vi "TestProcess.vi"(0 "VI Reference In":refnum<vi>, 5 "Wash Option":string, 7 "Car Position":u8=1, 9 "Elapsed Time":dbl=5.0, 11 "error in":errorcluster, 13 "Same Position?":bool) -> (4 "VI Reference Out":refnum<vi>, 15 "error out":errorcluster)   [LabVIEW 2016, in "CarWashTest.lvlib"]
doc: "Test Process function"
uses:
  CarWashTest.lvlib
  APIs/Assert/AssertControlValue/False.vi
  APIs/Assert/AssertControlValue/True.vi
  APIs/Stimulus/ControlValue/SetValueAuto.vi
  APIs/Assert/AssertControlValue/Equal.vi
  APIs/Assert/AssertControlValue/AlmostEqual.vi
  <vilib>/addons/_JKI Toolkits/Caraya/classes/Test/Test.lvclass
  Drona.lvlib
  APIs/Assert/AssertControlValue/AssertControlValue.lvlib
  APIs/Stimulus/ControlValue/ControlValue.lvlib
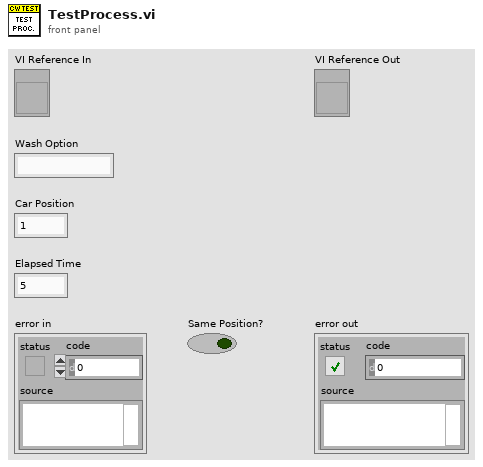
[diagram p1: front panel]
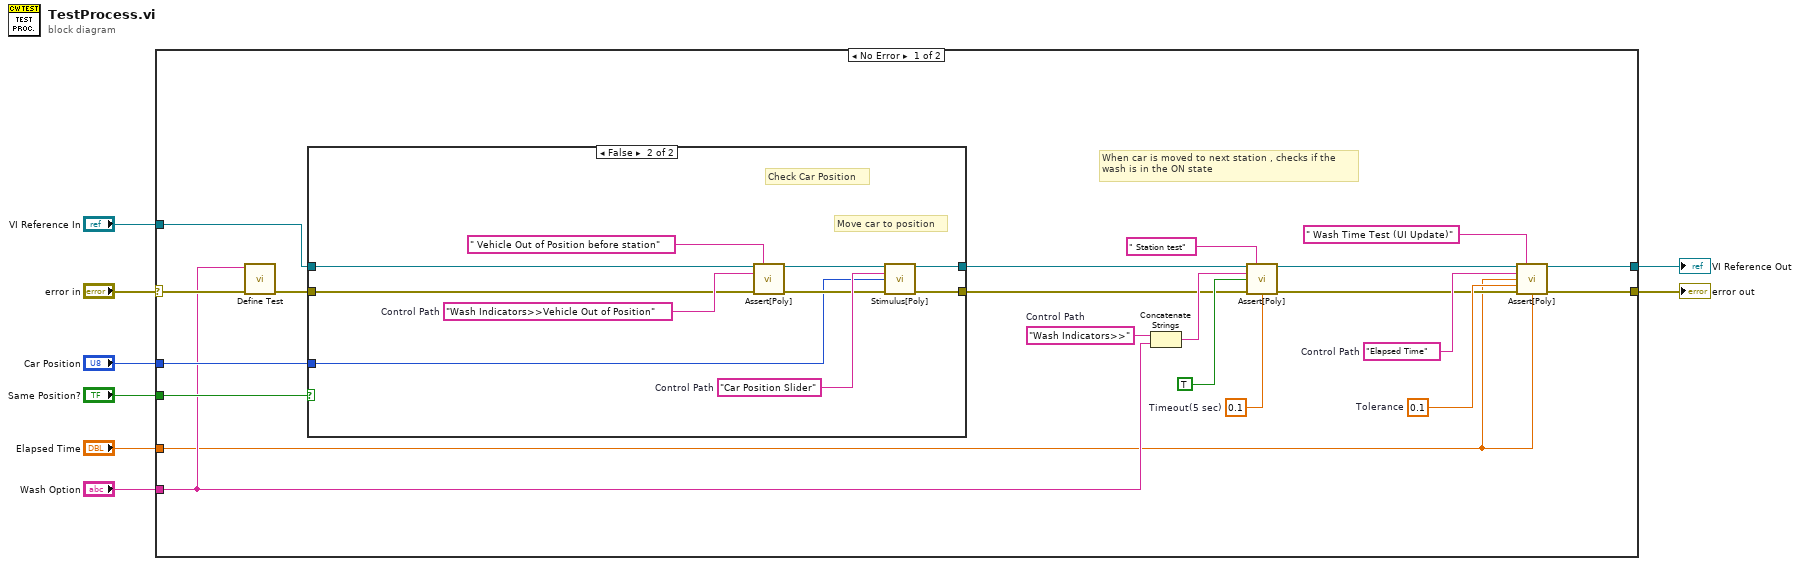
[diagram p0: block diagram]
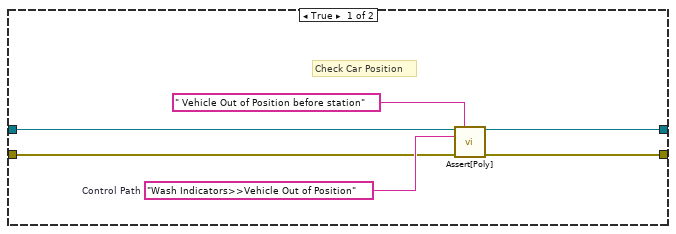
[diagram p2: hidden frame]
diagram:
  n1 = case shown="No Error" "error in" {
    selector: "error in" -> [w29 w46]
    tunnel: "VI Reference In" -> [w15 w47]
    tunnel: "Same Position?" -> [w14 _]
    tunnel: "Car Position" -> [w13 _]
    tunnel: [w12 w46] -> w4
    tunnel: [w11 w47] -> w3
    tunnel: "Wash Option" -> [w10 _]
    tunnel: "Elapsed Time" -> [w9 _]
    frame No Error {
      w20 = "Wash Indicators>>"  # Control Path
      w25 = 0.1  # Timeout(5 sec)
      w23 = 0.1  # Tolerance
      w24 = "Elapsed Time"  # Control Path
      # "When car is moved to next station , checks if the\nwash is in the ON state"
      n2 = call <vilib>:"Define Test.vi"("error in (no error)"=w29, "Label (VI Title)"=w10) -> ("error out"=w16:errorcluster)  [unwired: 8 in, 1 out]
      n3 = case shown="False" w14 {
        tunnel: [w32 w45] -> w17
        tunnel: [w31 w44] -> w21
        tunnel: w15 -> [w34 w41]
        tunnel: w16 -> [w33 w39]
        tunnel: w13 -> [_ w37]
        frame True {
          w35 = "Wash Indicators>>Vehicle Out of Position"  # Control Path
          # "Check Car Position"
          n4 = call-poly "Assert[Poly].vi"("VI Reference In"=w34, "Test Label"=" Vehicle Out of Position before station" ("Label"), "Control Path"=w35, "Error In"=w33) -> ("VI Reference Out"=w31:refnum<vi>, "Error Out"=w32:errorcluster)  [unwired: 9 in, 1 out]
        }
        frame False {
          w42 = "Wash Indicators>>Vehicle Out of Position"  # Control Path
          w43 = "Car Position Slider"  # Control Path
          # "Move car to position"
          # "Check Car Position"
          n5 = call-poly "Assert[Poly].vi"("VI Reference In"=w41, "Test Label"=" Vehicle Out of Position before station" ("Label"), "Control Path"=w42, "Error In"=w39) -> ("VI Reference Out"=w40:refnum<vi>, "Error Out"=w38:errorcluster)  [unwired: 9 in, 1 out]
          n6 = call-poly "Stimulus[Poly].vi"("VI Reference In"=w40, "Control Path"=w43, "Value (Signaling)"=w37, "error in"=w38) -> ("VI Reference Out"=w44:refnum<vi>, "error out"=w45:errorcluster)  [unwired: 10 in]
        }
      }
      n7 = Concatenate Strings(w20, w10) -> (w19:string)
      n8 = call-poly "Assert[Poly].vi"("VI Reference In"=w21, "Test Label"=" Station test" ("Label"), "Control Path"=w19, "Control Value"=TRUE, "Error In"=w17, "Timeout(5 sec)"=w25) -> ("VI Reference Out"=w22:refnum<vi>, "Error Out"=w18:errorcluster)  [unwired: 7 in, 1 out]
      n9 = call-poly "Assert[Poly].vi"("VI Reference In"=w22, "Test Label"=" Wash Time Test (UI Update)" ("Label"), "Control Path"=w24, "Control Value"=w9, "Tolerance"=w23, "Error In"=w18, "Timeout(5 sec)"=w9) -> ("VI Reference Out"=w11:refnum<vi>, "Error Out"=w12:errorcluster)  [unwired: 6 in, 1 out]
    }
    frame Error {
    }
  }
  "error out" <- w4
  "VI Reference Out" <- w3
